vi "Check Writer Backpressure.vi"(8 "error in (no error)":errorcluster, 10 "Timeout (ms)":i32, 11 "CIF_CIPC_Chn in":refnum<class "CIF_CIPC_Chn.lvclass">) -> (0 "error out":errorcluster, 2 "timed out?":bool)   [LabVIEW 2021, in "CIF_CIPC_Chn.lvclass"]
uses:
  CIF_CIPC_Chn.lvclass
  CIF_CIPC_Chn.lvclass/CIF_CIPC_Chn.ctl
  7796537b-0e69-421b-96bb-30a861203fb6.vi
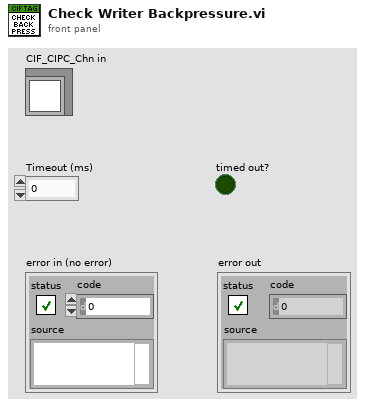
[diagram p1: front panel]
types:
  T1 = typedef "CIF_CIPC_Chn.lvclass/Buffer Configuration Data.ctl" = cluster{"Total Size":u32, "Read Size":u32, "Read Offset":u32, "CIPC BP References":T2, "CIPC Backpressure Names":T3, "Override CIPC Name":string, "Encoder Data":string}
  T2 = typedef "CIF_NI_CIPC.lvlib/Backpressure References.ctl" = cluster{"CIPC Reference":u64, "CIPC BP Reference":u64}
  T3 = typedef "CIF_NI_CIPC.lvlib/Backpressure Names.ctl" = cluster{"CIPC Name":string, "CIPC BP Name":string}
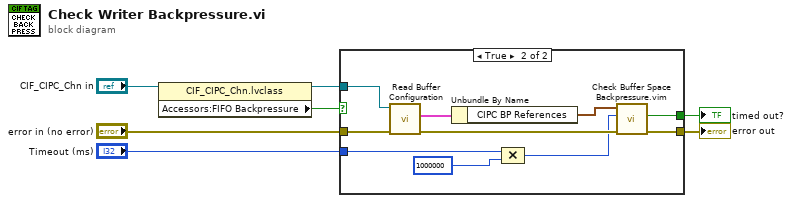
[diagram p0: block diagram]
diagram:
  n1 = property class="CIF_CIPC_Chn.lvclass"(reference="CIF_CIPC_Chn in") -> (reference out=w6:refnum<class "CIF_CIPC_Chn.lvclass">, "Accessors:FIFO Backpressure"=w7:bool)  [unwired: 1 in, 1 out]
  n2 = case shown="True" w7 {
    tunnel: [w8 w9] -> w2
    tunnel: "error in (no error)" -> [w8 w17]
    tunnel: w6 -> [_ w18]
    tunnel: [_ w13] -> w1
    tunnel: "Timeout (ms)" -> [_ w12]
    frame False {
    }
    frame True {
      n3 = call "Read Buffer Configuration.vi"("error in (no error)"=w17, "CIF_CIPC_Chn in"=w18) -> ("error out"=w14:errorcluster, "Buffer Configuration"=w16:T1)  [unwired: 7 in, 1 out]
      n4 = Unbundle By Name(w16) -> ("CIPC BP References"=w15:T2)
      n5 = Compound Arithmetic op=MULTIPLY(w12, 1000000 ("value")) -> (w10:i32)
      n6 = call "Check Buffer Space Backpressure.vim"("error in (no error)"=w14, "Timeout (ns)"=w10, "CIPC BP References in"=w15) -> ("error out"=w9:errorcluster, "Timeout"=w13:bool)  [unwired: 6 in, 1 out]
    }
  }
  "error out" <- w2
  "timed out?" <- w1
